vi "mupSetVarValue_Array.vi"(8 "error in (no error)":errorcluster, 10 "varValue":dbl[](array[numeric]), 11 "varPtr in":u64) -> (0 "error out":errorcluster, 3 "varPtr out":u64)   [LabVIEW 2015, in "mupLib.lvlib"]
doc: "Set the values of the bulk mode defined variable at the specified memory location.\n\nUse the address returned by the <b>mupDefineVar_Array</b> function as the input to <b>varAddr</b>.\n\n<b>Make sure that the varValue array is the same size as the array that was used for variable definition.</b>"
uses:
  mupLib.lvlib
panel:
  # "Set the values of the bulk mode defined variable at the specified memory location.\n\nUse the address returned by the mupDefineVar_Array function as the input to varAddr.\n\nMake sure that the varValue array is the same size as the array that was used for variable definition."
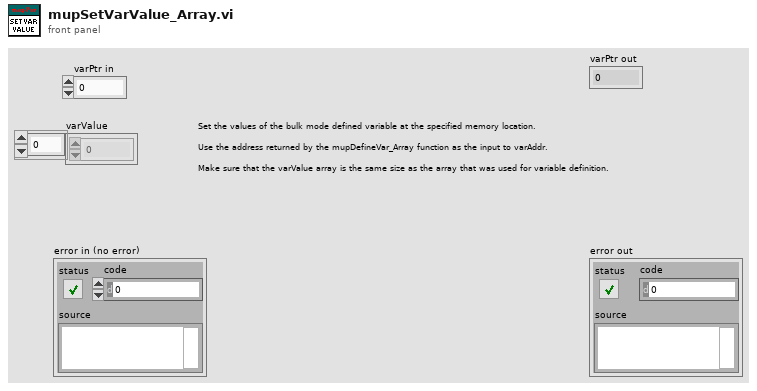
[diagram p1: front panel]
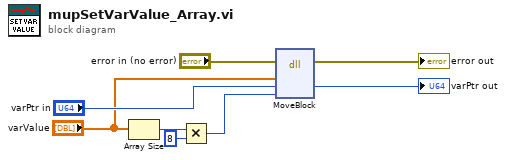
[diagram p0: block diagram]
diagram:
  n1 = Array Size(array="varValue") -> (size(s)=w8:i32)
  n2 = Multiply(x=w8, y=8) -> (x*y=w2:i32)
  n3 = dll-call lib="LabVIEW" fn="MoveBlock"(error in="error in (no error)", "ps"="varValue", "pd"="varPtr in", "size"=w2) -> (error out=→"error out":errorcluster, "pd"=→"varPtr out":u64)  [unwired: 5 in, 1 out]
